vi "Configure Secured TCP Client.vi"(4 "Read Mode (Immediate)":T1(ring)=enum."Immediate", 6 "timeout ms":i32=5000, 7 "Hostname":string="localhost", 8 "error in (no error)":errorcluster, 9 "Server X.509 Certificate":path, 10 "remote port (443)":u16=443, 11 "address (localhost)":string="localhost") -> (0 "error out":errorcluster, 2 "Ready for SSL":bool, 3 "Secured TCP Connection":refnum<class "Connection.TCP-TLS.lvclass">)   [LabVIEW 2020, in "Connection.TCP-TLS.lvclass"]
doc: "Creates a new TLS secured TCP-connection.\n\n<b>address</b>: IP-address or hostname of the server to connect to.\n<b>Hostname</b>: Hostname of the server certificate (PEM file).\nIn normal use cases the <b>address</b> and <b>Hostname</b> have the same input.\n\n---\nDeprecated -- kept for backward compatibility\nUse the \"Configure Secured TCP Client (Advanced)\" method instead."
uses:
  Connection.TCP-TLS.lvclass
  C:/Program Files (x86)/National Instruments/LabVIEW 2020/vi.lib/LabVIEW Open Source Project/MQTT TCP Connection/MQTT_TCP/Connection/TCPConnection.lvclass
  C:/Program Files (x86)/National Instruments/LabVIEW 2020/vi.lib/LabVIEW Open Source Project/Connection/Connection/Connection.lvclass
  Connection.TCP-TLS.lvclass/Connection.TCP-TLS.ctl
  <vilib>/LabVIEW Open Source Project/MQTT TCP Connection/MQTT_TCP/Connection/TCPConnection.lvclass/TCPConnection.ctl
  <vilib>/LabVIEW Open Source Project/Connection/Connection/Connection.lvclass/Connection.ctl
  <vilib>/LabVIEW Open Source Project/MQTT TCP Connection/MQTT_TCP/Connection/TCPConnection.lvclass
  <vilib>/LabVIEW Open Source Project/Connection/Connection/Connection.lvclass
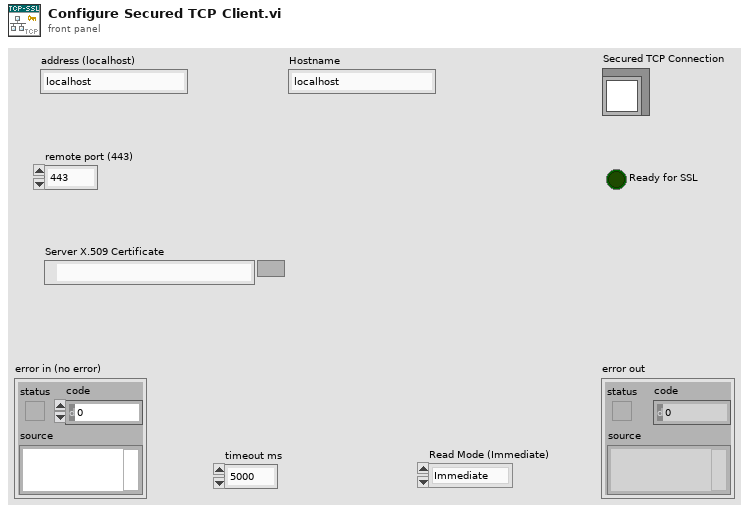
[diagram p1: front panel]
types:
  T1 = enum16{"Standard", "Buffered", "CRLF", "Immediate"}
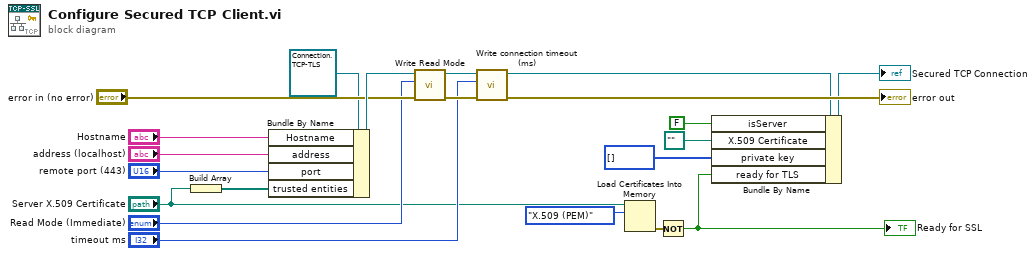
[diagram p0: block diagram]
diagram:
  n1 = Build Array("Server X.509 Certificate") -> (w4:path[])
  n2 = Bundle By Name(cluster=refnum<class "Connection.TCP-TLS.lvclass"> refnum ("Connection.TCP-TLS in"), "Hostname"="Hostname", "address"="address (localhost)", "port"="remote port (443)", "trusted entities"=w4) -> (w20:refnum<class "Connection.TCP-TLS.lvclass">)
  n3 = call <vilib>:"Write Read Mode.vi"("error in (no error)"="error in (no error)", "Read Mode"="Read Mode (Immediate)", "TCPConnection in"=w20) -> ("error out"=w19:errorcluster, "TCPConnection"=w21:refnum<class "Connection.TCP-TLS.lvclass">)  [unwired: 7 in]
  n4 = call <vilib>:"Write connection timeout (ms).vi"("error in (no error)"=w19, "connection timeout (ms)"="timeout ms", "Connection in"=w21) -> ("error out"=→"error out":errorcluster, "Connection out"=w8:refnum<class "Connection.TCP-TLS.lvclass">)  [unwired: 7 in]
  n5 = Load Certificates Into Memory(10:enum32{"X.509 (PEM)"}."X.509 (PEM)" ("format"), 11:"Server X.509 Certificate") -> (0:w10:errorcluster)  [unwired: 1 in, 1 out]
  n6 = Not(x=w10) -> (.not. x?=w1:bool)
  "Ready for SSL" <- w1
  n7 = Bundle By Name(cluster=w8, "isServer"=FALSE, "X.509 Certificate"=path "" ("Self.X.509 Certificate"), "private key"=u8[] [], "ready for TLS"=w1) -> (→"Secured TCP Connection":refnum<class "Connection.TCP-TLS.lvclass">)
